vi "CO check Ant Pol.vi"(8 "error in (no error)":errorcluster caption="에러 입력(에러 없음)", 9 "Mast Index":i32=1, 10 "Antenna Pol":enum16{"H", "V"}(ring), 11 "Instrument Manager 입력":refnum<class "Instrument Manager.lvclass">) -> (0 "error out":errorcluster caption="에러 출력", 2 "needChange?":bool, 3 "Instrument Manager 출력":refnum<class "Instrument Manager.lvclass">)   [LabVIEW 2023, in "Instrument Manager.lvclass"]
uses:
  Instrument Manager.lvclass
  Module/Turn Table and Mast Control/Class/CO3000/CO3000.lvclass
  Module/Turn Table and Mast Control/Interface Class/Mast/Interface - Mast.lvclass
  Instrument Manager.lvclass/Instrument Manager.ctl
  C:/Users/HCT-3320/Documents/Instrument Manger/Module/Turn Table and Mast Control/Class/CO3000/CO3000.lvclass
  C:/Users/HCT-3320/Documents/Instrument Manger/Module/Turn Table and Mast Control/Interface Class/Mast/Interface - Mast.lvclass
  C:/Users/HCT-3320/Documents/Instrument Manger/Module/Turn Table and Mast Control/Interface Class/Turn Table/Interface - Turn Table.lvclass
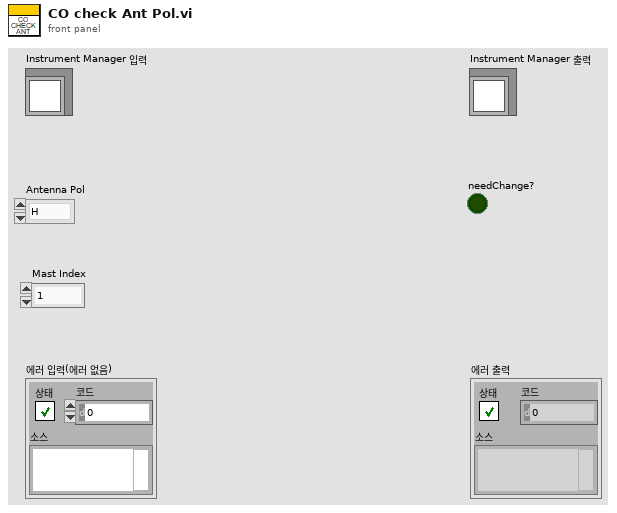
[diagram p1: front panel]
types:
  T1 = cluster{"Anritsu Call Box":refnum<class "Anritsu Call Box.lvclass">, "Spectrum Analyzer":refnum<class "Interface_Spectrum.lvclass">, "RF Switch Box":refnum<class "RF Filter Box.lvclass">, "Turn Table":refnum<class "Interface - Turn Table.lvclass">, "Mast":refnum<class "Interface - Mast.lvclass">, "3D Controller":refnum<class "Interface_3D Controller.lvclass">}
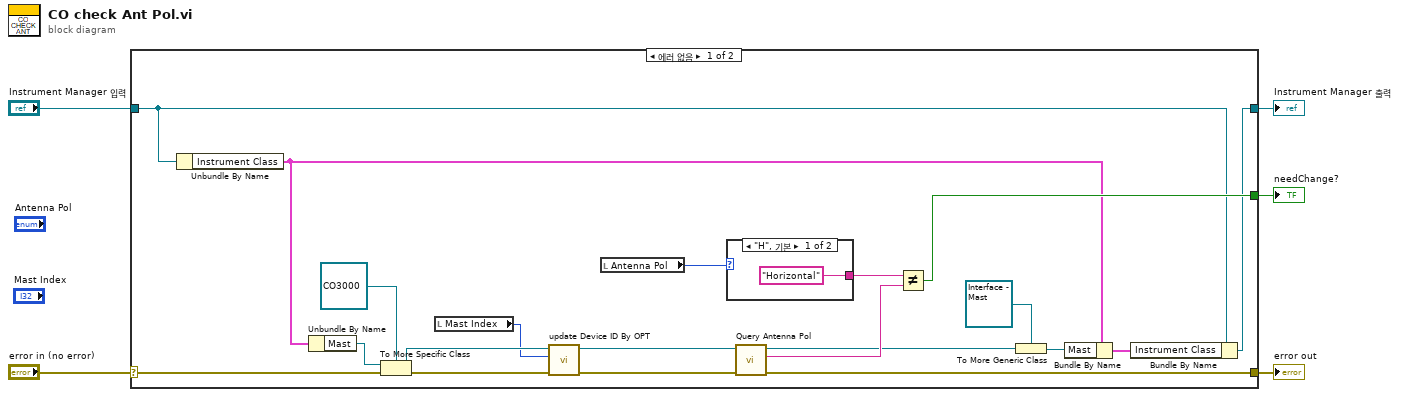
[diagram p0: block diagram]
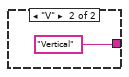
[diagram p2: hidden frame]
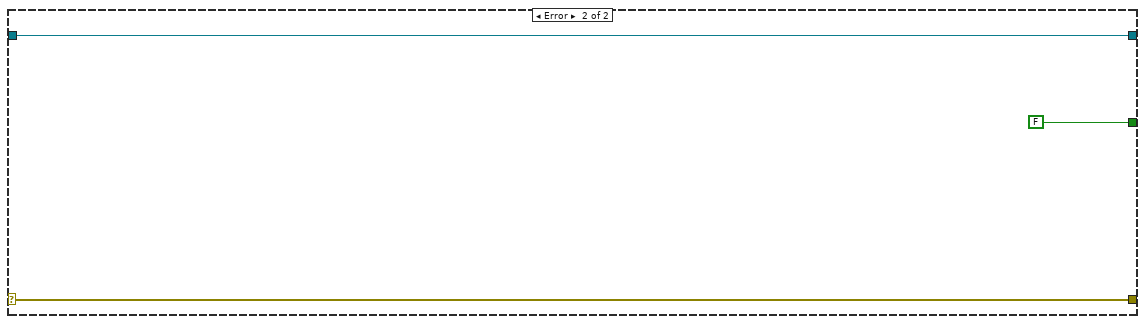
[diagram p3: hidden frame]
diagram:
  n1 = case shown="에러 없음" "error in (no error)" {
    selector: "error in (no error)" -> [w22 w30]
    tunnel: [w8 w30] -> w4
    tunnel: [w9 w29] -> w2
    tunnel: "Instrument Manager 입력" -> [w11 w29]
    tunnel: [w16 FALSE] -> w1
    frame No Error {
      n2 = Unbundle By Name(w11) -> ("Instrument Class"=w15:T1)
      n3 = Unbundle By Name(w15) -> ("Mast"=w23:refnum<class "Interface - Mast.lvclass">)
      n4 = To More Specific Class(target class=refnum<class "CO3000.lvclass"> refnum ("Turn Table and Mast.lvlib:CO3000.lvclass"), reference=w23, error in=w22) -> (specific class reference=w20:refnum<class "CO3000.lvclass">, error out=w21:errorcluster)
      n5 = local read "Mast Index"() -> (w7:i32)
      n6 = call "update Device ID By OPT.vi"("error in (no error)"=w21, "Mast Index"=w7, "CO3000 in"=w20) -> ("error out"=w17:errorcluster, "CO3000 out"=w18:refnum<class "CO3000.lvclass">)  [unwired: 5 in, 2 out]
      n7 = local read "Antenna Pol"() -> (w6:enum16{"H", "V"})
      n8 = case shown="\"H\", 기본" w6 {
        tunnel: ["Horizontal" "Vertical"] -> w24
        frame "H", Default {
        }
        frame "V" {
        }
      }
      n9 = call-dynamic "Query Antenna Pol.vi"("error in (no error)"=w17, "CO3000 in"=w18) -> ("error out"=w8:errorcluster, "Antenna Pol"=w25:string, "CO3000 out"=w14:refnum<class "CO3000.lvclass">)  [unwired: 7 in]
      n10 = Not Equal?(x=w24, y=w25) -> (x != y?=w16:bool)
      n11 = To More Generic Class(target class=refnum<class "Interface - Mast.lvclass"> refnum ("Turn Table and Mast.lvlib:Interface - Mast.lvclass"), reference=w14) -> (generic class reference=w13:refnum<class "Interface - Mast.lvclass">)
      n12 = Bundle By Name(cluster=w15, "Mast"=w13) -> (w10:T1)
      n13 = Bundle By Name(cluster=w11, "Instrument Class"=w10) -> (w9:refnum<class "Instrument Manager.lvclass">)
    }
    frame Error {
    }
  }
  "error out" <- w4
  "Instrument Manager 출력" <- w2
  "needChange?" <- w1
